vi "Test MQTT-3.14.4-1.vi"(8 "error in (no error)":errorcluster, 11 "Connection Config":refnum<class "Connection.lvclass">) -> (0 "error out":errorcluster, 3 "Connection Config dup":refnum<class "Connection.lvclass">)   [LabVIEW 2013]
uses:
  <vilib>/LabVIEW Open Source Project/MQTT Control Packets/Control Packets/CONNACK/Connect Return Code -- enum.ctl
  <vilib>/LabVIEW Open Source Project/MQTT Connection/MQTT_Connection/Connection/Connection.lvclass
  <vilib>/addons/_JKI Toolkits/Caraya/classes/Test/Test.lvclass
  <vilib>/LabVIEW Open Source Project/MQTT Client/Client class/Client.lvclass
  <vilib>/addons/_JKI Toolkits/Caraya/classes/Assert/Assert.lvclass
  <vilib>/LabVIEW Open Source Project/MQTT Control Packets/Control Packets/DISCONNECT/DISCONNECT.lvclass
  <vilib>/LabVIEW Open Source Project/MQTT Connection/MQTT_Base/Base Class/MQTT_Base.lvclass
  <vilib>/LabVIEW Open Source Project/MQTT Control Packets/Control Packets/CONNACK/CONNACK.lvclass
panel:
  out "Return Code":T1=enum."Server Unavailable"
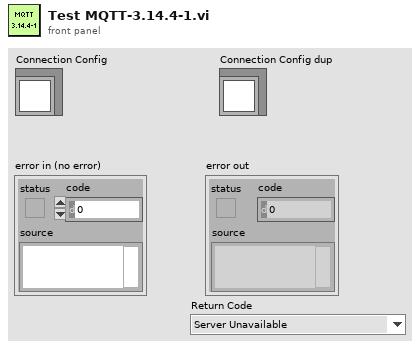
[diagram p1: front panel]
types:
  T1 = typedef "MQTT_Control_Packets.lvlib/CONNACK.lvclass/Connect Return Code -- enum.ctl" = enum16{"Connection accepted", "Unacceptable protocol version", "Identifier Rejected", "Server Unavailable", "Bad Username or Password", "Not Authorized"}
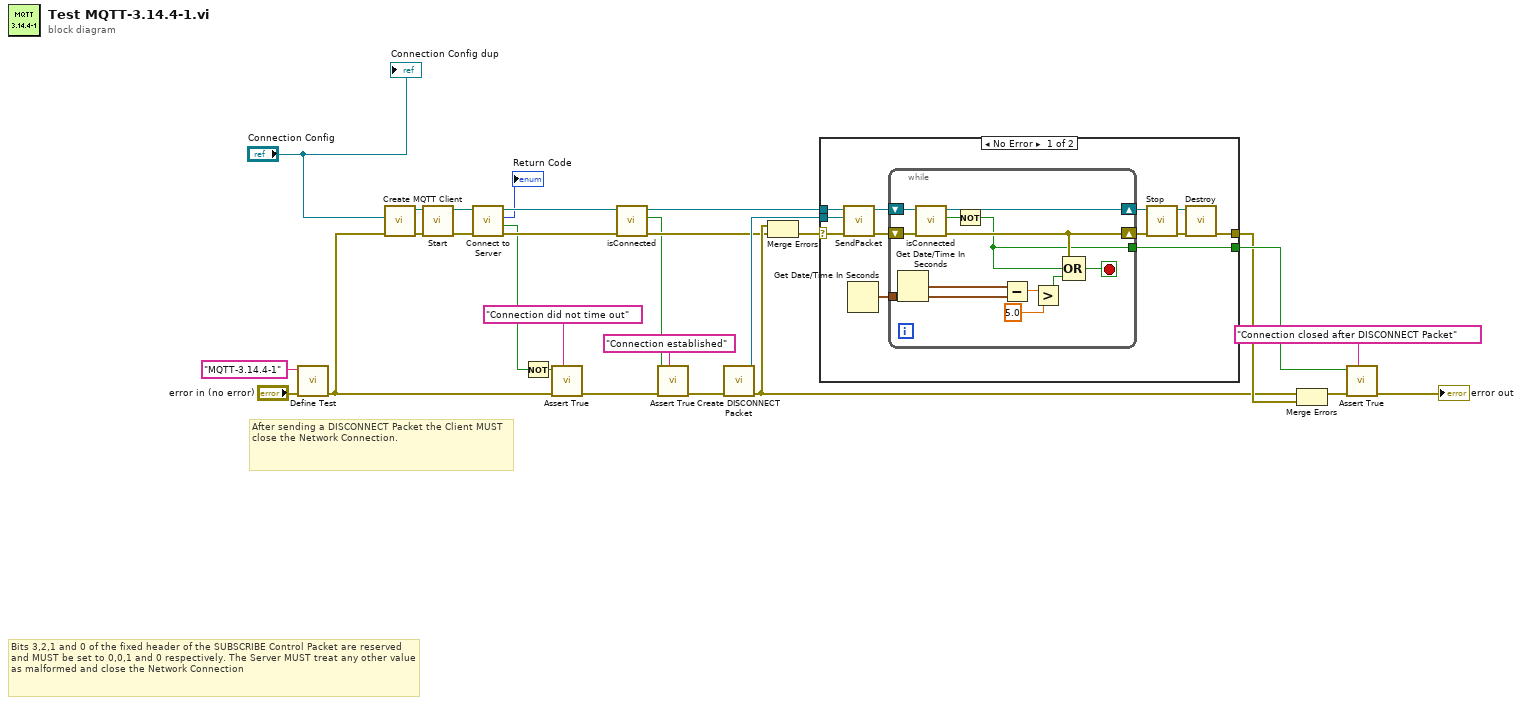
[diagram p0: block diagram]
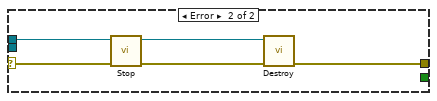
[diagram p2: hidden frame]
diagram:
  # "After sending a DISCONNECT Packet the Client MUST close the Network Connection."
  # "Bits 3,2,1 and 0 of the fixed header of the SUBSCRIBE Control Packet are reserved and MUST be set to 0,0,1 and 0 respectively. The Server MUST treat any other value as malformed and close the Network Connection"
  n1 = call <vilib>:"Define Test.vi"("error in (no error)"="error in (no error)", "Label (VI Title)"="MQTT-3.14.4-1") -> ("error out"=w6:errorcluster)  [unwired: 9 in]
  n2 = call <vilib>:"Create MQTT Client.vi"("error in (no error)"=w6, "Connection Configuration"="Connection Config") -> ("error out"=w18:errorcluster, "Client out"=w20:refnum<class "Client.lvclass">)  [unwired: 8 in]
  n3 = call <vilib>:"Start.vi"("error in (no error)"=w18, "MQTT_Base in"=w20) -> ("error out"=w17:errorcluster, "MQTT_Base out"=w19:refnum<class "Client.lvclass">)  [unwired: 7 in, 1 out]
  n4 = call <vilib>:"Connect to Server.vi"("error in (no error)"=w17, "Client in"=w19) -> ("error out"=w14:errorcluster, "timed out"=w4:bool, "Return Code"=→"Return Code":T1, "Client out"=w12:refnum<class "Client.lvclass">)  [unwired: 6 in]
  n5 = Not(x=w4) -> (.not. x?=w3:bool)
  n6 = call <vilib>:"Assert True.vi"("Label"="Connection did not time out", "error in (no error)"=w6, "True?"=w3) -> ("error out"=w5:errorcluster)  [unwired: 8 in]
  n7 = call <vilib>:"isConnected.vi"("error in (no error)"=w14, "Client in"=w12) -> ("error out"=w13:errorcluster, "connected"=w8:bool, "Client out"=w11:refnum<class "Client.lvclass">)  [unwired: 7 in]
  n8 = call <vilib>:"Assert True.vi"("Label"="Connection established", "error in (no error)"=w5, "True?"=w8) -> ("error out"=w9:errorcluster)  [unwired: 8 in]
  n9 = call <vilib>:"Create DISCONNECT Packet.vi"("error in (no error)"=w9) -> ("error out"=w15:errorcluster, "DISCONNECT"=w16:refnum<class "DISCONNECT.lvclass">)  [unwired: 8 in, 1 out]
  n10 = Merge Errors(w15, w13) -> (w21:errorcluster)
  n11 = case shown="No Error" w21 {
    selector: w21 -> [w38 w54]
    tunnel: w11 -> [w39 w56]
    tunnel: [w40 w57] -> w22
    tunnel: [w34 _] -> w24
    tunnel: w16 -> [w37 _]
    frame No Error {
      n12 = call <vilib>:"SendPacket.vi"("error in (no error)"=w38, "ControlPacket"=w37, "Client in"=w39) -> ("error out"=w35:errorcluster, "Client out"=w36:refnum<class "Client.lvclass">)  [unwired: 6 in, 1 out]
      n13 = Get Date/Time In Seconds() -> (seconds since 1Jan1904=w33:timestamp)
      n14 = while {
        shift-right: [w49] -> w30
        shift-left: w35 -> [w50]
        shift-right: [w51] -> w32
        shift-left: w36 -> [w52]
        tunnel: [w46] -> w34
        tunnel: w33 -> [w41]
        stop <- w48 stop-if-true
        n15 = Get Date/Time In Seconds() -> (seconds since 1Jan1904=w45:timestamp)
        n16 = call <vilib>:"isConnected.vi"("error in (no error)"=w50, "Client in"=w52) -> ("error out"=w49:errorcluster, "connected"=w47:bool, "Client out"=w51:refnum<class "Client.lvclass">)  [unwired: 7 in]
        n17 = Not(x=w47) -> (.not. x?=w46:bool)
        n18 = Subtract(x=w45, y=w41) -> (x-y=w44:dbl)
        n19 = Greater?(x=w44, y=5.0) -> (0:w42:bool)
        n20 = Compound Arithmetic op=OR(w49, w46, w42) -> (w48:bool)
      }
      n21 = call <vilib>:"Stop.vi"("error in (no error)"=w30, "MQTT_Base in"=w32) -> ("error out"=w29:errorcluster, "MQTT_Base out"=w31:refnum<class "Client.lvclass">)  [unwired: 7 in, 1 out]
      n22 = call <vilib>:"Destroy.vi"("error in (no error)"=w29, "MQTT_Base in"=w31) -> ("error out"=w40:errorcluster)  [unwired: 8 in, 1 out]
    }
    frame Error {
      n23 = call <vilib>:"Stop.vi"("error in (no error)"=w54, "MQTT_Base in"=w56) -> ("error out"=w53:errorcluster, "MQTT_Base out"=w55:refnum<class "Client.lvclass">)  [unwired: 7 in, 1 out]
      n24 = call <vilib>:"Destroy.vi"("error in (no error)"=w53, "MQTT_Base in"=w55) -> ("error out"=w57:errorcluster)  [unwired: 8 in, 1 out]
    }
  }
  n25 = Merge Errors(w15, w22) -> (w23:errorcluster)
  n26 = call <vilib>:"Assert True.vi"("Label"="Connection closed after DISCONNECT Packet", "error in (no error)"=w23, "True?"=w24) -> ("error out"=→"error out":errorcluster)  [unwired: 8 in]
  "Connection Config dup" <- "Connection Config"
